vi "UE_Stop_Requested.vi"(1 "global_fault":bool, 2 "operator_stop":bool) -> (0 "must_stop":bool)   [LabVIEW 2026]
doc: "INTENT: Combine operator stop request and global fault request. INPUTS: operator_stop (bool), global_fault (bool). OUTPUTS: must_stop (bool). DESIGN CONSTRAINT: Safety action must not wait for this VI or an ordinary executor loop. REQUIREMENTS: SRS-F-015. No physical hardware side effects. Acceptance requires native LabVIEW compilation and behavioral testing."
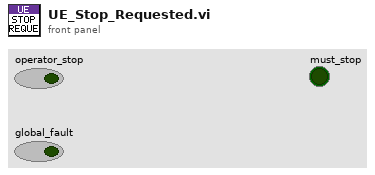
[diagram p1: front panel]
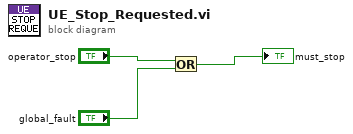
[diagram p0: block diagram]
diagram:
  n1 = Or(x="operator_stop", y="global_fault") -> (x .or. y?=→"must_stop":bool)
